vi "Native_GetForTerminals.vi"() -> ()   [LabVIEW 2024]
panel:
  out "error out":errorcluster caption="错误输出"
  out "counter_id":u32
  in  "counter_id type":u32
  out "count_id":u32
  in  "count_id type":u32
  in  "for_id":u32
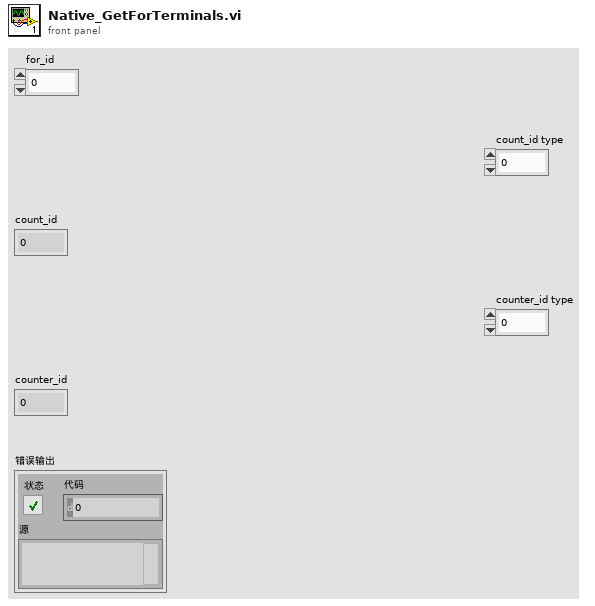
[diagram p1: front panel]
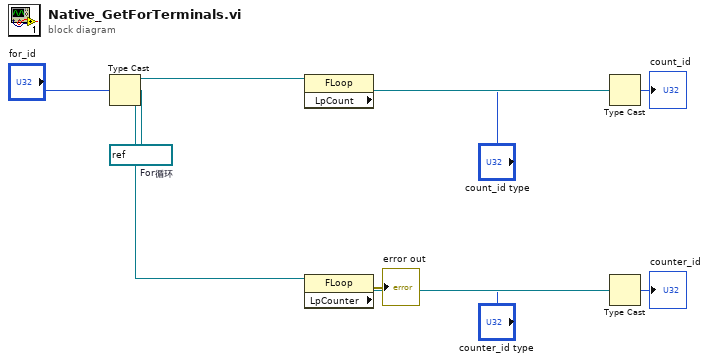
[diagram p0: block diagram]
diagram:
  w9 = refnum<vi> refnum  # For循环
  n1 = Type Cast ("强制类型转换")(type=w9, x="for_id") -> (*(type *) &x=w8:refnum<vi>)
  n2 = property on="属性节点" class="FLoop"(reference=w8) -> ("LpCount"=w7:refnum<vi>)  [unwired: 1 in, 2 out]
  n3 = property on="属性节点" class="FLoop"(reference=w8) -> (error out=→"error out":errorcluster, "LpCounter"=w4:refnum<vi>)  [unwired: 1 in, 1 out]
  n4 = Type Cast ("强制类型转换")(type="count_id type", x=w7) -> (*(type *) &x=→"count_id":u32)
  n5 = Type Cast ("强制类型转换")(type="counter_id type", x=w4) -> (*(type *) &x=→"counter_id":u32)
